vi "RemoteVI Window Frame Encode.vi"(0 "id":u32, 5 "seq":u32, 7 "width":u16, 9 "height":u16, 11 "rects":cluster{"x":i16, "y":i16, "png":string}[](array[cluster])) -> (4 "message":string)   [LabVIEW 2020, in "RemoteVI.lvlib"]
doc: "Encodes one RemoteVI protocol v2 WINDOW FRAME message (docs/protocol.md section 7) - the picture of another window of the application (a dialog, a file dialog, a subVI panel) with the same dirty-rectangle encoding as FRAME. Layout, all integers big-endian: 0x52, 0x03, window id U32, seq U32 (shared with FRAME), width U16, height U16, rect count U16, then per rect x I16, y I16, png length U32 and the png bytes. Pure function, cannot fail. Reference: encodeWindowFrame() in tools\\lib\\protocol.mjs."
uses:
  RemoteVI.lvlib
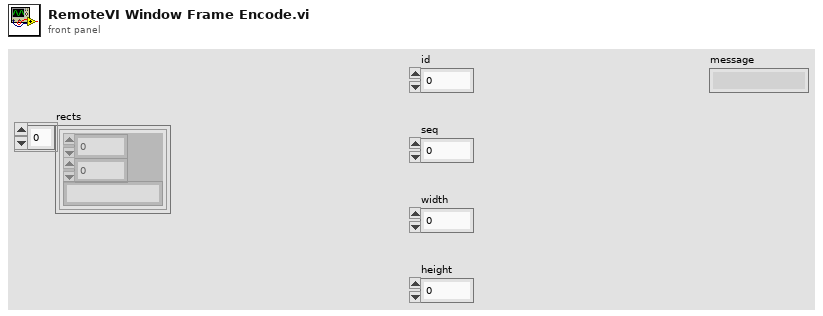
[diagram p1: front panel]
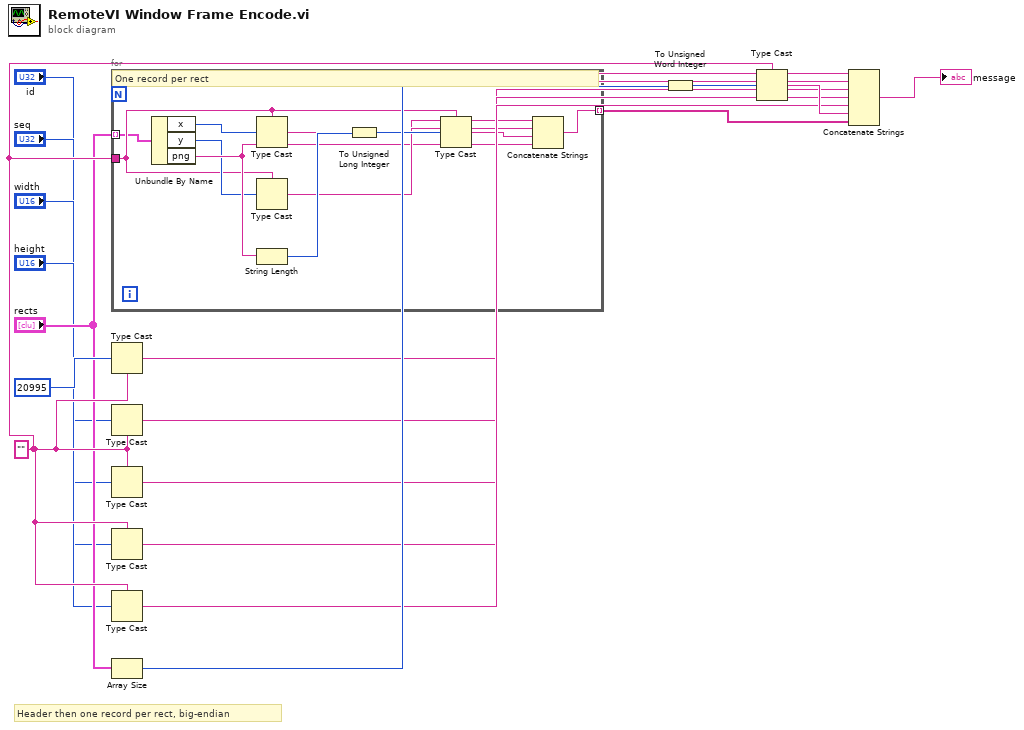
[diagram p0: block diagram]
diagram:
  w7 = ""
  # "Header then one record per rect, big-endian"
  n1 = for {
    tunnel: "rects" -> [w18] mode=indexing
    tunnel: w7 -> [w19]
    tunnel: [w28] -> w16 mode=indexing
    # "One record per rect"
    n2 = Unbundle By Name(w18) -> ("x"=w20:i16, "y"=w21:i16, "png"=w22:string)
    n3 = Type Cast(type=w19, x=w20) -> (*(type *) &x=w23:string)
    n4 = Type Cast(type=w19, x=w21) -> (*(type *) &x=w24:string)
    n5 = String Length(string=w22) -> (length=w25:i32)
    n6 = To Unsigned Long Integer(number=w25) -> (unsigned 32bit integer=w26:u32)
    n7 = Type Cast(type=w19, x=w26) -> (*(type *) &x=w27:string)
    n8 = Concatenate Strings(w23, w24, w27, w22) -> (w28:string)
  }
  n9 = Type Cast(type=w7, x=u16 20995) -> (*(type *) &x=w8:string)
  n10 = Type Cast(type=w7, x="id") -> (*(type *) &x=w9:string)
  n11 = Type Cast(type=w7, x="seq") -> (*(type *) &x=w10:string)
  n12 = Type Cast(type=w7, x="width") -> (*(type *) &x=w11:string)
  n13 = Type Cast(type=w7, x="height") -> (*(type *) &x=w12:string)
  n14 = Array Size(array="rects") -> (size(s)=w13:i32)
  n15 = To Unsigned Word Integer(number=w13) -> (unsigned 16bit integer=w14:u16)
  n16 = Type Cast(type=w7, x=w14) -> (*(type *) &x=w15:string)
  n17 = Concatenate Strings(w8, w9, w10, w11, w12, w15, w16) -> (→"message":string)
